vi "GDSLvClass_GetLibraryItemFromPath.vi"(0 "Library Refnum In":refnum<vi>, 1 "VINames":path, 5 "error in (no error)":errorcluster, 8 "CreateThePhysicalFolderIfPossible(True)":bool=TRUE, 9 "VirtualFolderScope":T1(array[ring])) -> (14 "Item Refnum Out":refnum<vi>, 19 "error out":errorcluster)   [LabVIEW 2020]
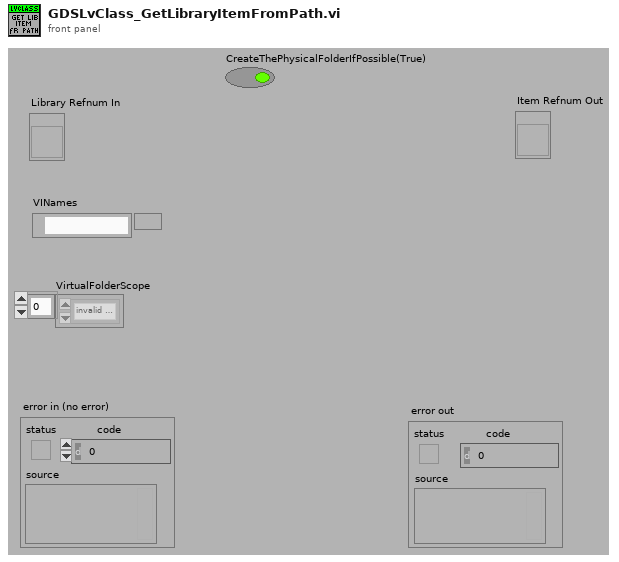
[diagram p1: front panel]
types:
  T1 = enum32{"invalid scope", "public", "private", "protected", "community"}[]
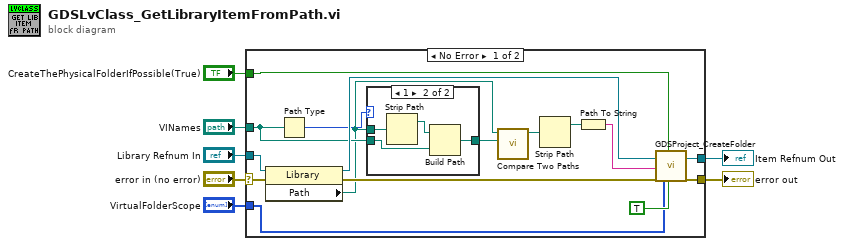
[diagram p0: block diagram]
diagram:
  n1 = case shown="No Error" "error in (no error)" {
    selector: "error in (no error)" -> [w22 w29]
    tunnel: [w14 w29] -> w6
    tunnel: "Library Refnum In" -> [w23 _]
    tunnel: [w15 _] -> w4
    tunnel: "VINames" -> [w10 _]
    tunnel: "CreateThePhysicalFolderIfPossible(True)" -> [w13 _]
    tunnel: "VirtualFolderScope" -> [w8 _]
    frame No Error {
      n2 = property class="Library"(reference=w23, error in=w22) -> (reference out=w20:refnum<vi>, error out=w19:errorcluster, "Path"=w9:path)
      n3 = Path Type(1:w10) -> (0:w12:i16)
      n4 = case shown="1" w12 {
        tunnel: w10 -> [w24 w26]
        tunnel: w9 -> [_ w28]
        tunnel: [w24 w25] -> w11
        frame 0, Default {
        }
        frame 1 {
          n5 = Strip Path(path=w28) -> (stripped path=w27:path)  [unwired: 1 out]
          n6 = Build Path(base path=w27, name or relative path=w26) -> (appended path=w25:path)
        }
      }
      n7 = call <vilib>:"Compare Two Paths.vi"("Path 2"=w11, "Path 1"=w9) -> ("Relative Path from 1 to 2"=w21:path)  [unwired: 6 in, 3 out]
      n8 = Strip Path(path=w21) -> (stripped path=w18:path)  [unwired: 1 out]
      n9 = Path To String(path=w18) -> (string=w17:string)
      n10 = call "GDSProject_CreateFolder.vi"("Project Item To Create Folder Below(Use MyComputer if not wired)"=w20, "FolderName"=w17, "error in (no error)"=w19, "FolderScope"=w8, "CreateThePhysicalFolderIfPossible(False)"=w13, "GuessFolderScope(False)"=TRUE) -> ("ItemOut"=w15:refnum<vi>, "error out"=w14:errorcluster)  [unwired: 10 in, 2 out]
    }
    frame Error {
    }
  }
  "Item Refnum Out" <- w4
  "error out" <- w6
